vi "MPExxx_get_per.vi"(0 "VISA session":refnum<visa-resource-name>, 1 "error in (no error)":errorcluster) -> (2 "dup VISA session":refnum<visa-resource-name>, 3 "Period Setting":string, 4 "error out":errorcluster)   [LabVIEW 2012]
doc: "This VI form retrieves the current period setting."
uses:
  MPExxx Globals.gbl
panel:
  # "MAGNA-POWER"
  # "Electronics"
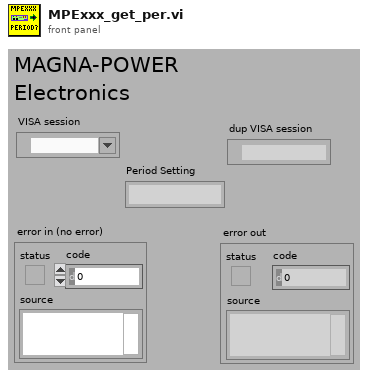
[diagram p1: front panel]
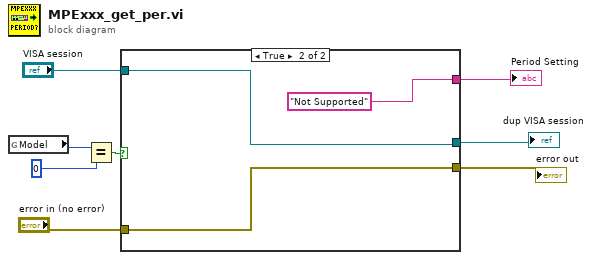
[diagram p0: block diagram]
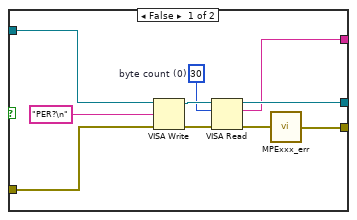
[diagram p2: hidden frame]
diagram:
  n1 = global read "MPExxx Globals.gbl" "Model"() -> (w6:u8)
  n2 = Equal?(x=w6, y=0) -> (x = y?=w8:bool)
  n3 = case shown="True" w8 {
    tunnel: [w13 w20] -> w2
    tunnel: [w12 w19] -> w1
    tunnel: [w11 "Not Supported"] -> w3
    tunnel: "VISA session" -> [w10 w20]
    tunnel: "error in (no error)" -> [w9 w19]
    frame False {
      w16 = u32 30  # byte count (0)
      n4 = VISA Write(VISA resource name=w10, write buffer="PER?\n", error in (no error)=w9) -> (VISA resource name out=w17:refnum<visa-resource-name>, error out=w15:errorcluster)  [unwired: 1 out]
      n5 = VISA Read(VISA resource name=w17, byte count=w16, error in (no error)=w15) -> (VISA resource name out=w13:refnum<visa-resource-name>, read buffer=w11:string, error out=w14:errorcluster)  [unwired: 1 out]
      n6 = call "MPExxx_err.vi"("error in (no error)"=w14) -> ("error out"=w12:errorcluster)
    }
    frame True {
    }
  }
  "Period Setting" <- w3
  "error out" <- w1
  "dup VISA session" <- w2
